vi "PicoScope3000aGetStreamingValues.vi"(9 "deviceIndex":u16, 11 "error in":errorcluster) -> (0 "Start Index":u32, 1 "Trigger":cluster{bool, "triggeredAt (Total samples)":u32}, 3 "error out":errorcluster, 4 "Number of Samples":i32, 5 "ready":i16, 6 "Auto Stopped":bool)   [LabVIEW 2010]
doc: "This VI is used in streaming mode to get the latest values from the driver. It should be called in a loop after the oscilloscope has been set up using PicoScope3000aSettings.vi and streaming has been started by calling PicoScope3000aStartStreaming.vi. The VI outputs the number of samples available and the start index of these samples in the array output by PicoScope3000aStartStreaming.vi."
uses:
  ps3000aWrap.dll
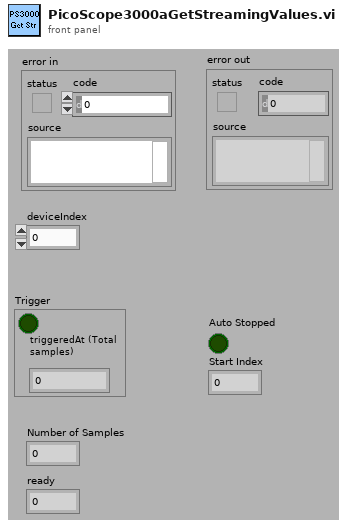
[diagram p1: front panel]
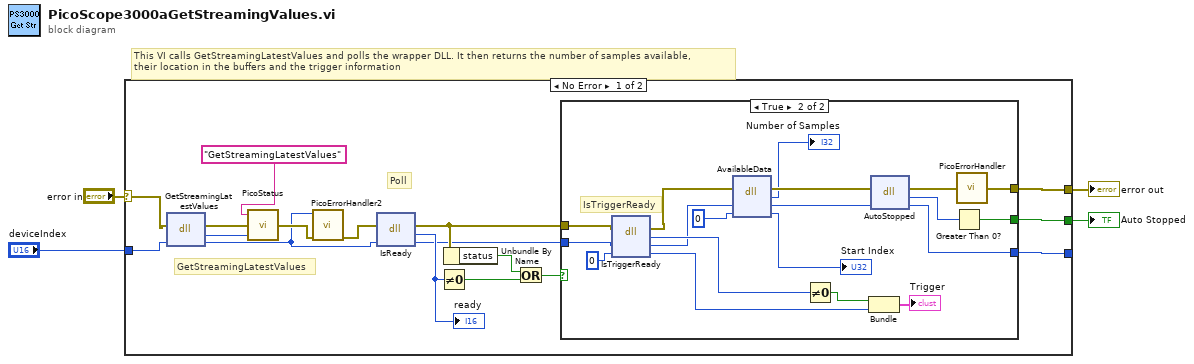
[diagram p0: block diagram]
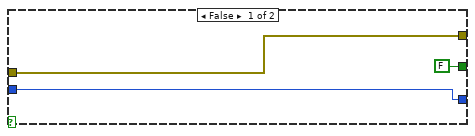
[diagram p2: hidden frame]
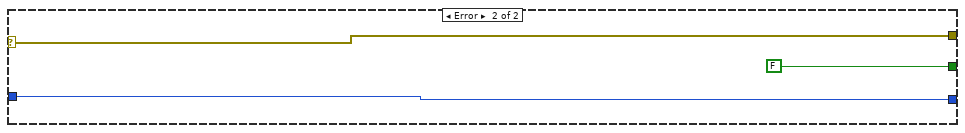
[diagram p3: hidden frame]
diagram:
  # "This VI calls GetStreamingLatestValues and polls the wrapper DLL. It then returns the number of samples available, \ntheir location in the buffers and the trigger information"
  n1 = case shown="No Error" "error in" {
    selector: "error in" -> [w13 w46]
    tunnel: [w21 w46] -> w3
    tunnel: [w20 w44] -> _
    tunnel: [w19 FALSE] -> w2
    tunnel: "deviceIndex" -> [w5 w44]
    frame No Error {
      # "Poll"
      # "GetStreamingLatestValues"
      n2 = dll-call lib="ps3000aWrap.dll" fn="GetStreamingLatestValues" ("PS5000.dll:_ps5000SetDataBuffer@16")(error in=w13, "deviceIndex"=w5) -> (error out=w12:errorcluster, "PICO_STATUS"=w11:u32, "deviceIndex"=w9:u16)  [unwired: 2 in, 1 out]
      n3 = call "PicoStatus.vi"("PICO STATUS"=w11, "error in"=w12, "source"="GetStreamingLatestValues") -> ("error out"=w15:errorcluster)
      n4 = call "PicoErrorHandler2.vi"("error in (no error)"=w15, "handle In"=w9) -> ("error out"=w10:errorcluster)  [unwired: 9 in]
      n5 = dll-call lib="ps3000aWrap.dll" fn="IsReady" ("PS5000.dll:_ps5000SetDataBuffer@16")(error in=w10, "DeviceIndex"=w9) -> (error out=w8:errorcluster, "ready"=w7:i16, "DeviceIndex"=w6:u16)  [unwired: 2 in, 1 out]
      "ready" <- w7
      n6 = Not Equal To 0?(x=w7) -> (x != 0?=w17:bool)
      n7 = Unbundle By Name(w8) -> ("status"=w18:bool)
      n8 = Or(x=w18, y=w17) -> (x .or. y?=w14:bool)
      n9 = case shown="True" w14 {
        tunnel: [w24 w43] -> w21
        tunnel: w6 -> [w23 w38]
        tunnel: w8 -> [w24 w39]
        tunnel: [w23 w32] -> w20
        tunnel: [FALSE w40] -> w19
        frame False {
        }
        frame True {
          # "IsTriggerReady"
          n10 = dll-call lib="ps3000aWrap.dll" fn="IsTriggerReady" ("PS5000.dll:_ps5000SetDataBuffer@16")(error in=w39, "deviceIndex"=w38, "triggeredAt"=u32 0) -> (error out=w31:errorcluster, "triggered"=w35:i16, "deviceIndex"=w30:u16, "triggeredAt"=w36:u32)  [unwired: 2 in, 1 out]
          n11 = dll-call lib="ps3000aWrap.dll" fn="AvailableData" ("PS5000.dll:_ps5000Stop@4")(error in=w31, "deviceIndex"=w30, "startIndex"=u32 0) -> (error out=w28:errorcluster, "numSamples"=→"Number of Samples":i32, "deviceIndex"=w27:u16, "startIndex"=→"Start Index":u32)  [unwired: 2 in, 1 out]
          n12 = Not Equal To 0?(x=w35) -> (x != 0?=w42:bool)
          n13 = Bundle(w42, "triggeredAt"=w36) -> (→"Trigger":cluster{bool, "triggeredAt":u32})  [unwired: 1 in]
          n14 = dll-call lib="ps3000aWrap.dll" fn="AutoStopped"(error in=w28, "deviceIndex"=w27) -> (error out=w34:errorcluster, "AutoStopped"=w33:i16, "deviceIndex"=w32:u16)  [unwired: 2 in, 1 out]
          n15 = Greater Than 0?(x=w33) -> (x > 0?=w40:bool)
          n16 = call "PicoErrorHandler.vi"("error in"=w34) -> ("error out"=w43:errorcluster)
        }
      }
    }
    frame Error {
    }
  }
  "error out" <- w3
  "Auto Stopped" <- w2
